vi "05b-multiple_functions.vi"() -> ()   [LabVIEW 2018, in "LV2Julia_examples.lvlib"]
uses:
  LV2Julia_examples.lvlib
  LV2Julia_core/VIs/Server or client state.ctl
  LV2Julia_core/VIs/detailed error info.ctl
  LV2Julia_core/VIs/StackFrame.ctl
  LV2Julia_core/VIs/Commands.ctl
  b50b62fa-0ed7-4d6a-8a9d-aa54acf293b0.vi
  b50b62fa-0ed7-4d6a-8a9d-aa54acf293b0.vi/52173681-d551-446d-9107-ca47c949d000.vi
  b50b62fa-0ed7-4d6a-8a9d-aa54acf293b0.vi/52173681-d551-446d-9107-ca47c949d000.vi/cc902bbf-88f4-4796-bad4-1a41209f7faa.vi
  b50b62fa-0ed7-4d6a-8a9d-aa54acf293b0.vi/52173681-d551-446d-9107-ca47c949d000.vi/e4202884-77c7-4b96-ba0a-fabb5cdf4261.vi
  b50b62fa-0ed7-4d6a-8a9d-aa54acf293b0.vi/52173681-d551-446d-9107-ca47c949d000.vi/0c284a69-23ec-4246-87e0-e46ed227f5dc.vi
  LV2Julia_core/VIs/jl-scripts path.vi
  LV2Julia_core/VIs/check ID validity.vi
  LV2Julia_core/VIs/bindata_descr to JSON.vi
  LV2Julia_core/VIs/check cluster field names.vi
  LV2Julia_core/VIs/concat JSON.vi
  LV2Julia_core/VIs/build request.vi
  LV2Julia_core/VIs/Parse server response.vi
  LV2Julia_core/VIs/log jl exceptions.vi
  LV2Julia_core/LV2Julia_core.lvlib
panel:
  in  "operation":u16(ring) items=["addition", "subtraction", "multiplication", "division", "conquer"]
  in  "operands":cluster{"x":dbl, "y":dbl}={"x"=2.0, "y"=2.0}
  in  "next":bool
  out "result":dbl=nan
  out "detailed error info":T1
  out "current error":errorcluster
  out "final error":errorcluster
  out "short err code":u8
  in  "stop":bool
  out "ZMQ timeout":bool
  out "Julia script file path":path
  out "temporary script path":path
  out "Jl Server state":T3
  # "available functions loaded on start from the Julia server"
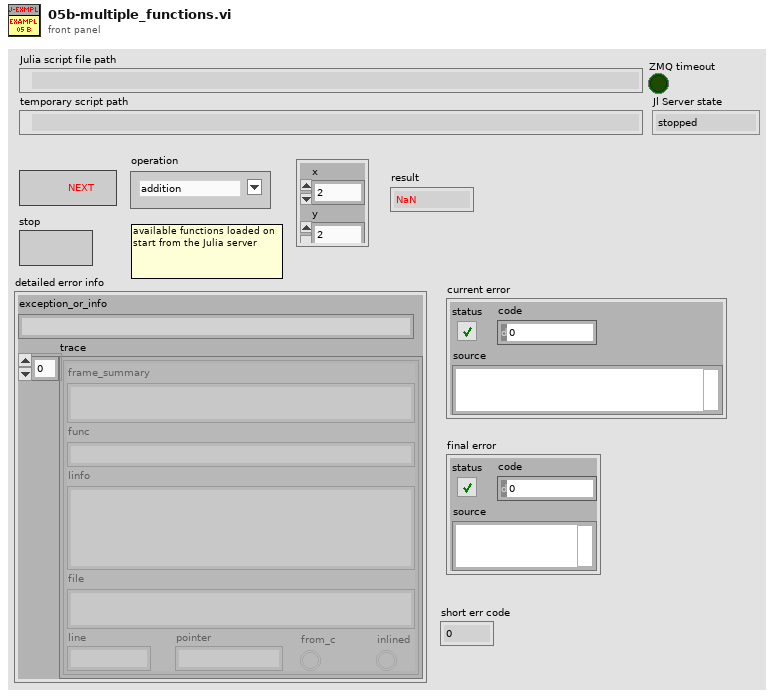
[diagram p1: front panel]
types:
  T1 = typedef "LV2Julia_core.lvlib/detailed error info.ctl" = cluster{"exception_or_info":string, "trace":T2[]}
  T2 = typedef "LV2Julia_core.lvlib/StackFrame.ctl" = cluster{"frame_summary":string, "func":string, "linfo":string, "file":string, "line":i32, "pointer":u64, "from_c":bool, "inlined":bool}
  T3 = typedef "LV2Julia_core.lvlib/Server or client state.ctl" = enum16{"stopped", "running", "unknown"}
  T4 = typedef "LV2Julia_core.lvlib/Commands.ctl" = enum16{"Start Jl-server & Init LV-client", "Send request & Get response ", "Stop Jl-server & Cleanup LV-client", "Cleanup LV-client", "Start Jl-server", "Stop Jl-server", "Init LV-Client", "Cleanup LV-Client", "(not allowed)", "Set LV Client state", "Set Jl Server state", "set ZMQ timeout", "read ZMQ timeout", "read-out state"}
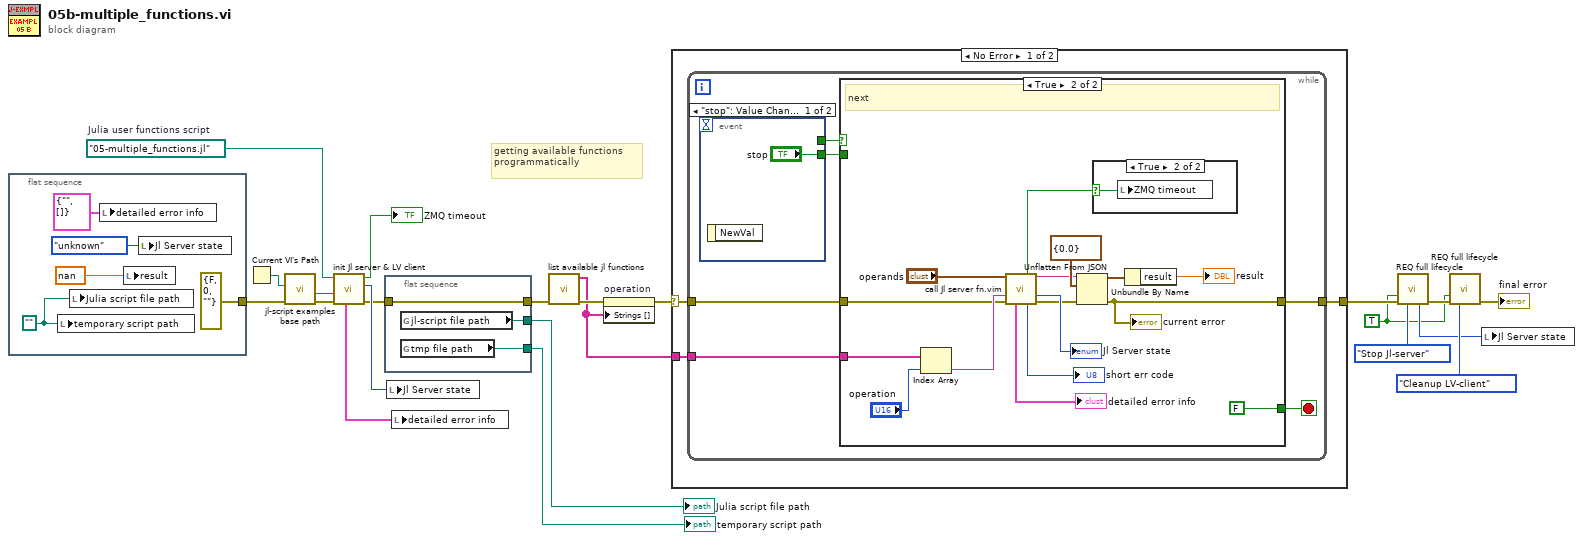
[diagram p0: block diagram]
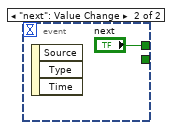
[diagram p2: hidden frame]
diagram:
  w9 = path "05-multiple_functions.jl"  # Julia user functions script
  w14 = TRUE ("Force command")
  # "getting available functions programmatically"
  n1 = flat-sequence {
    tunnel: [errorcluster {"status"=FALSE, "code"=0, "source"=""} ("error in (no error)")] -> w3
    frame #0 {
      w23 = path ""
      n2 = local write "temporary script path"(w23) -> ()
      n3 = local write "Julia script file path"(w23) -> ()
      n4 = local write "detailed error info"(T1 {"exception_or_info"="", "trace"=[]} ("detailed error info")) -> ()
      n5 = local write "result"(nan ("Server response")) -> ()
      n6 = local write "Jl Server state"(Server_or_client_state."unknown" ("Jl Server state out")) -> ()
    }
  }
  n7 = Current VI's Path() -> (path=w5:path)
  n8 = call "jl-script examples base path.vi"("error in (no error)"=w3, "calling example VI path"=w5) -> ("error out"=w4:errorcluster, "jl-script-examples base path"=w2:path)  [unwired: 8 in]
  n9 = call "init Jl server & LV client.vi"("error in (no error)"=w4, "Base path (not a path)"=w2, "Julia user functions script"=w9) -> ("error out"=w6:errorcluster, "Jl Server state out"=w7:T3, "timeout?"=→"ZMQ timeout":bool, "detailed error info"=w1:T1)  [unwired: 3 in, 2 out]
  n10 = flat-sequence {
    tunnel: [w30] -> w13
    tunnel: w6 -> [w30]
    tunnel: [w29] -> w16
    tunnel: [w28] -> w17
    frame #0 {
      n11 = global read "jl-scripts path.vi" "jl-script file path"() -> (w29:path)
      n12 = global read "jl-scripts path.vi" "tmp file path"() -> (w28:path)
    }
  }
  n13 = local write "Jl Server state"(w7) -> ()
  n14 = local write "detailed error info"(w1) -> ()
  n15 = call "list available jl functions.vi"("error in (no error)"=w13) -> ("error out"=w12:errorcluster, "ext_fns"=w10:string[])  [unwired: 4 in, 5 out]
  n16 = property on="operation" class="Ring (strict)"(error in=w12, "Strings []"=w10) -> (error out=w11:errorcluster)  [unwired: 1 in, 1 out]
  n17 = case shown="No Error" w11 {
    selector: w11 -> [w32 w61]
    tunnel: [w33 w61] -> w22
    tunnel: w10 -> [w31 _]
    frame No Error {
      n18 = while {
        tunnel: w32 -> [w38]
        tunnel: [w39] -> w33
        tunnel: w31 -> [w34]
        stop <- w36 stop-if-true
        n19 = event shown="[0] \"stop\": Value Change" {
          selector: _ -> [_ _]
          dyn-events: _ -> [_ _]
          timeout: _ -> [_ _]
          tunnel: [_ "next"] -> w37
          tunnel: ["stop" _] -> w35
          event "stop": Value Change {
            n20 = event-data() -> ()  [unwired: 1 in, 1 out]
          }
          event "next": Value Change {
            n21 = event-data() -> ()  [unwired: 1 in, 3 out]
          }
        }
        n22 = case shown="True" w37 {
          tunnel: [w43 w56] -> w39
          tunnel: w38 -> [w43 w50]
          tunnel: [w42 FALSE ("stop this VI only")] -> w36
          tunnel: w35 -> [w42 _]
          tunnel: w34 -> [_ w54]
          frame False {
            # "stop"
          }
          frame True {
            # "next"
            n23 = Index Array(array=w54, index="operation") -> (element=w51:string)
            n24 = call "call Jl server fn.vim"("Arguments 1"="operands", "fun2call"=w51, "error in (no error)"=w50) -> ("timeout?"=w47:bool, "JSON received"=w45:string, "Jl Server state out"=→"Jl Server state":T3, "detailed error info"=→"detailed error info":T1, "return code"=→"short err code":u8, "error out"=w48:errorcluster)  [unwired: 6 in, 1 out]
            n25 = Unflatten From JSON(JSON string=w45, type and defaults=cluster{"result":dbl} {"result"=0.0} ("parsed response"), error in (no error)=w48) -> (value=w58:cluster{"result":dbl}, error out=w56:errorcluster)  [unwired: 4 in]
            "current error" <- w56
            n26 = case shown="True" w47 {
              selector: w47 -> [_ w60]
              frame False {
              }
              frame True {
                n27 = local write "ZMQ timeout"(w60) -> ()
              }
            }
            n28 = Unbundle By Name(w58) -> ("result"=→"result":dbl)
          }
        }
      }
    }
    frame Error {
    }
  }
  n29 = call "REQ full lifecycle.vi"("Force command"=w14, "error in"=w22, "command"=Commands."Stop Jl-server") -> ("Jl Server state out"=w15:T3, "error out"=w20:errorcluster)  [unwired: 6 in, 5 out]
  n30 = call "REQ full lifecycle.vi"("Force command"=w14, "error in"=w20, "command"=Commands."Cleanup LV-client") -> ("error out"=→"final error":errorcluster)  [unwired: 6 in, 6 out]
  n31 = local write "Jl Server state"(w15) -> ()
  "temporary script path" <- w17
  "Julia script file path" <- w16
